vi "FX_BuildFrame.vi"(10 "Content":string, 11 "Command":string) -> (3 "Frame":string)   [LabVIEW 2026]
doc: "Use this template to build a VI to use as a subVI."
panel:
  # "ÕfÃ÷£º½M¾Ž³Ì…f¶¨·â°ü£ºSTX + ÃüÁî + ƒÈÈÝ + ETX + ºÍ\nÐ£òž¡£ºÍÐ£òž£½STX Ö®ááµ½ ETX µÄ¿‚ºÍÈ¡µÍ 8 Î»¡£"
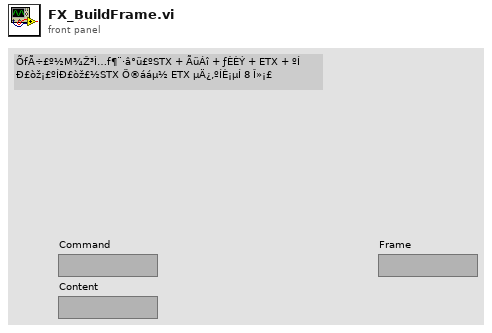
[diagram p1: front panel]
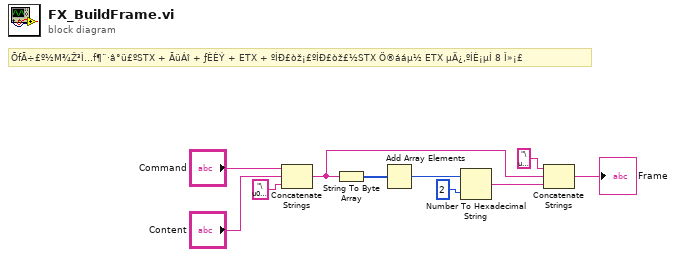
[diagram p0: block diagram]
diagram:
  # "ÕfÃ÷£º½M¾Ž³Ì…f¶¨·â°ü£ºSTX + ÃüÁî + ƒÈÈÝ + ETX + ºÍÐ£òž¡£ºÍÐ£òž£½STX Ö®ááµ½ ETX µÄ¿‚ºÍÈ¡µÍ 8 Î»¡£"
  n1 = Concatenate Strings("Command", "Content", "\u0003") -> (w7:string)
  n2 = String To Byte Array(string=w7) -> (unsigned byte array=w6:u8[])
  n3 = Add Array Elements(numeric array=w6) -> (sum=w5:u8)
  n4 = Number To Hexadecimal String(1:i16 2 ("width (-)"), 2:w5) -> (0:w2:string)
  n5 = Concatenate Strings("\u0002", w7, w2) -> (→"Frame":string)
